vi "Native_GetCaseInfo.vi"() -> ()   [LabVIEW 2024]
panel:
  out "error out":errorcluster caption="错误输出"
  out "selector_id":u32
  in  "selector_id type":u32
  out "frame_ids":u32[](array[numeric])
  in  "frame_ids type":u32
  in  "case_id":u32
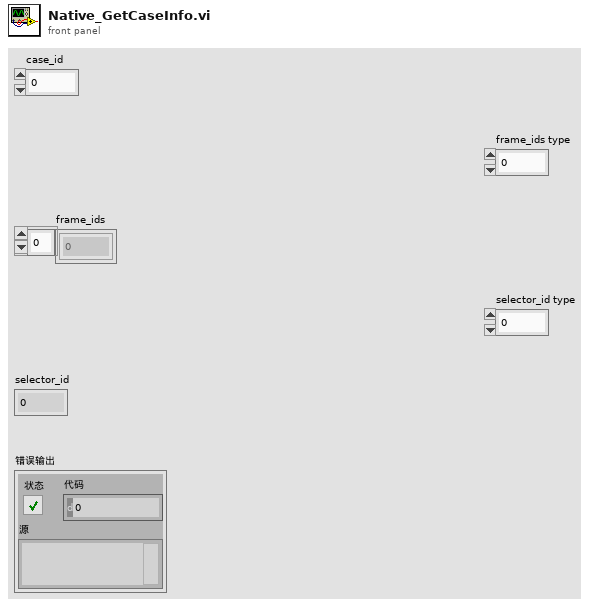
[diagram p1: front panel]
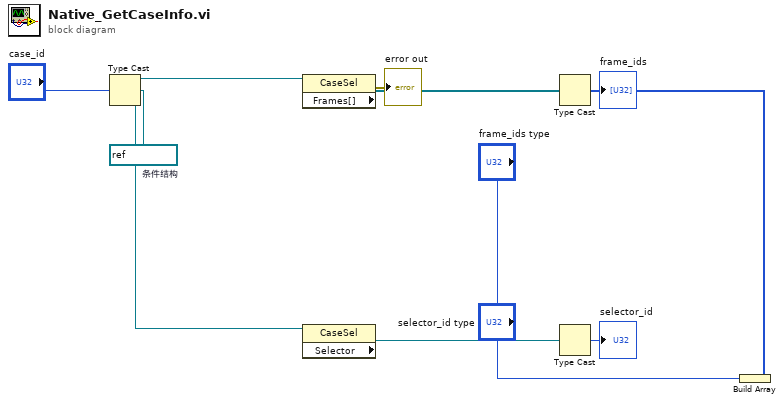
[diagram p0: block diagram]
diagram:
  w10 = refnum<vi> refnum  # 条件结构
  n1 = Type Cast ("强制类型转换")(type=w10, x="case_id") -> (*(type *) &x=w9:refnum<vi>)
  n2 = property on="属性节点" class="CaseSel"(reference=w9) -> (error out=→"error out":errorcluster, "Frames[]"=w8:refnum<vi>[])  [unwired: 1 in, 1 out]
  n3 = property on="属性节点" class="CaseSel"(reference=w9) -> ("Selector"=w4:refnum<vi>)  [unwired: 1 in, 2 out]
  n4 = Type Cast ("强制类型转换")(type="selector_id type", x=w4) -> (*(type *) &x=→"selector_id":u32)
  n5 = Build Array ("创建数组")("frame_ids type") -> (w6:u32[])
  n6 = Type Cast ("强制类型转换")(type=w6, x=w8) -> (*(type *) &x=→"frame_ids":u32[])
